vi "VIH HelpGen - Build Progress Info Window.vi"(6 "Mode (run1)":enum16{"start", "stop", "run1", "run2"}(ring)=enum."run1", 7 "Message":string, 8 "error in":errorcluster, 9 "# steps":i32, 10 "step idx":i32=-1, 11 "Cur path":path) -> (0 "error out":errorcluster)   [LabVIEW 2014]
doc: "::: VI Helpeks :::\nCopyright (c) 2000-2026 Konstantin Shifershteyn. All rights reserved."
uses:
  <vilib>/Platform/browser.llb/Open URL in Default Browser (path).vi
panel:
  in  "%OpenHelp":bool caption="Open Built Help"
  in  "%Explore":bool caption="Explore"
  out "errors":string
  in  "%ShowLog":bool caption="Open Build Log"
  out "progress info":string="1 of 1"
  out "Progress bar":i32(slide) scale=0.0..2.0
  out "State":string="Running..."
  out "Current path":string="file path..."
  in  "%Cancel":bool caption="Cancel"
  in  "%DONE":bool caption="Done"
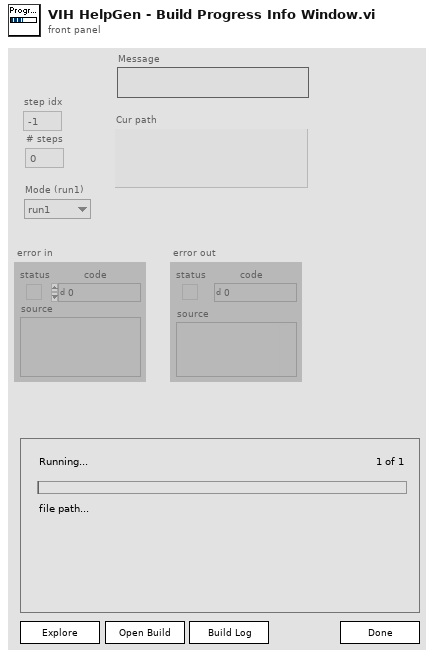
[diagram p1: front panel]
types:
  T1 = cluster{"Common path":path, "HTML File paths":path[], "CHM Path":path}
  T2 = enum8{"Enabled", "Disabled", "Disabled and Grayed Out"}
  T3 = cluster{"Selection Start":i32, "Selection End":i32}
  T4 = cluster{"Show Window":bool, "Show Progress":bool, "Generate HTML":bool, "Generate HHP":bool, "Generate CHM":bool}
  T5 = typedef "eventvkey.ctl" = enum16{"ASCII", "Enter", "Return", "Shift", "Ctrl", "Alt", "Cmd", "Opt", "Caps", "NumLock", "Clear", "Break", "Up", "Down", "Left", "Right", "Insert", "Delete", "Home", "End", "PageUp", "PageDown", "Escape", "Help", "Pause", "ScrollLock", "F1", "F2", "F3", "F4", "F5", "F6", "F7", "F8", "F9", "F10", "F11", "F12", "F13", "F14", "F15", "F16", "F17", "F18", "F19", "F20", "F21", "F22", "F23", "F24", "Play", "VolumeUp", "VolumeDown", "Mute", "Two Byte Char"}
  T6 = cluster{"Shift":bool, "Ctrl":bool, "Alt":bool, "Cmd":bool, "Opt":bool}
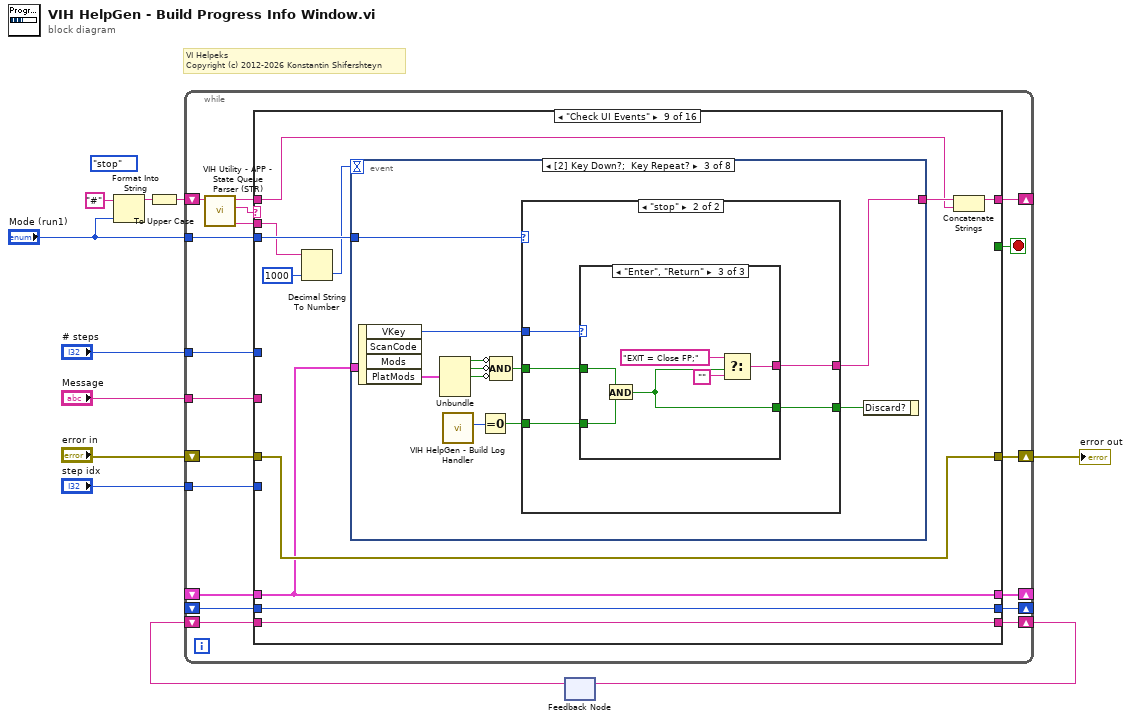
[diagram p0: block diagram]
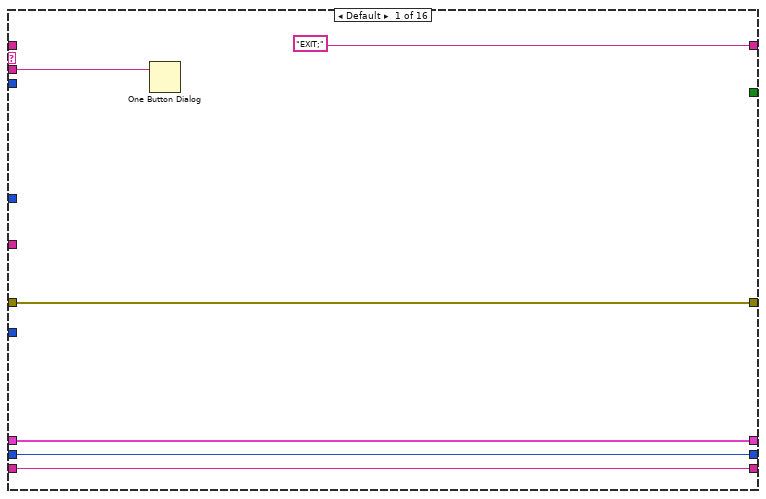
[diagram p2: hidden frame]
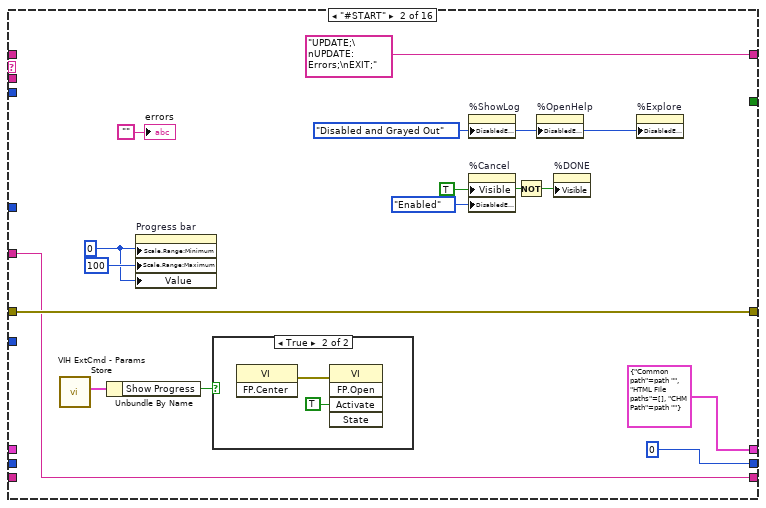
[diagram p3: hidden frame]
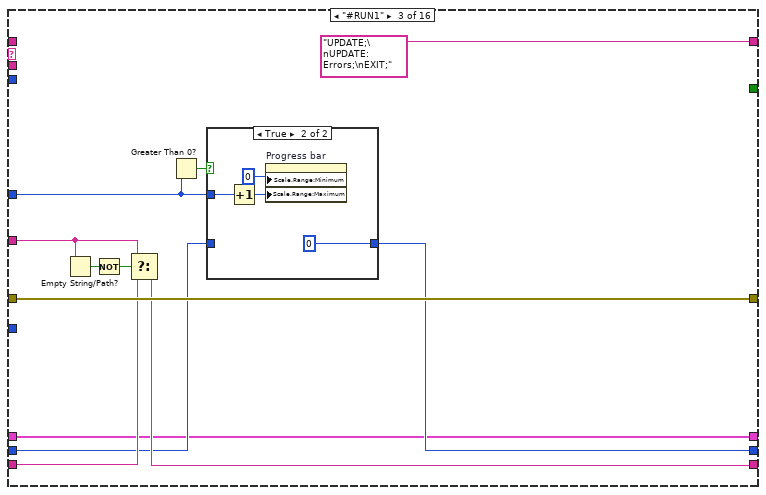
[diagram p5: hidden frame]
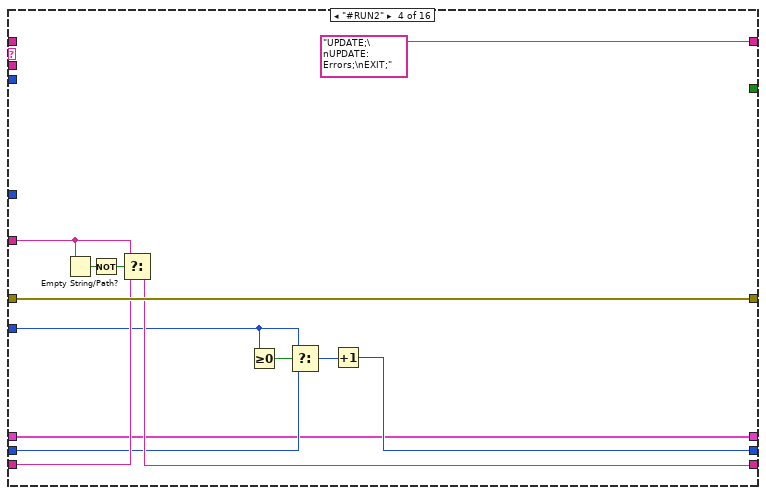
[diagram p7: hidden frame]
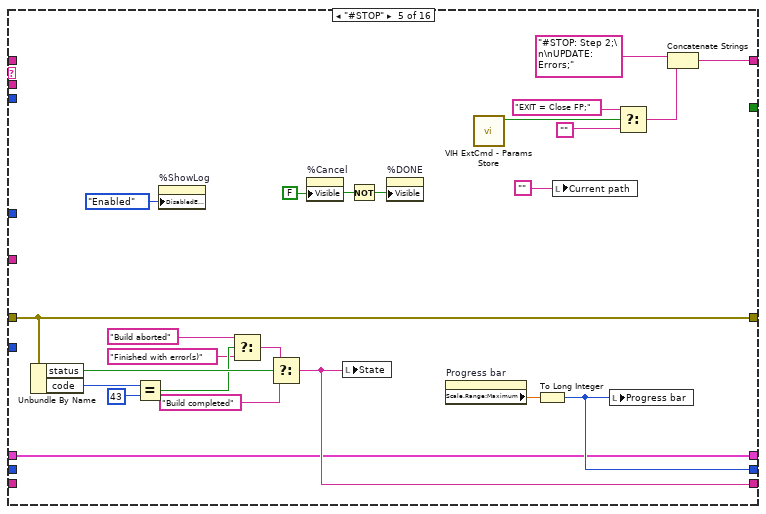
[diagram p8: hidden frame]
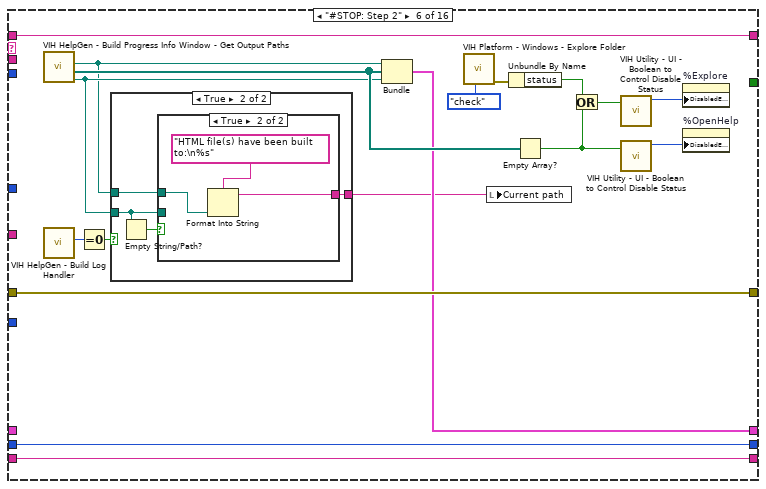
[diagram p9: hidden frame]
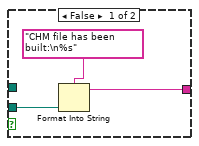
[diagram p11: hidden frame]
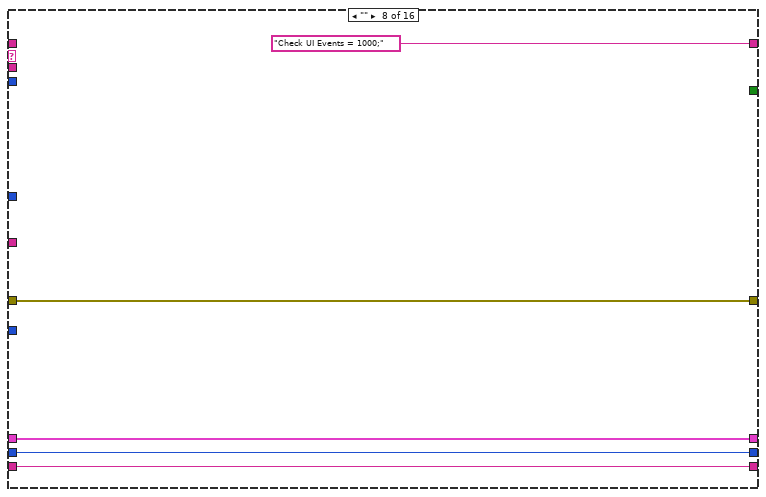
[diagram p13: hidden frame]
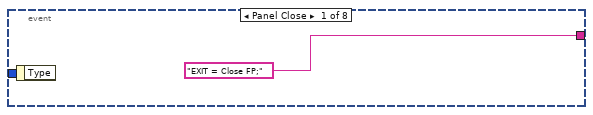
[diagram p14: hidden frame]
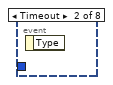
[diagram p15: hidden frame]
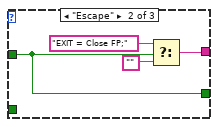
[diagram p18: hidden frame]
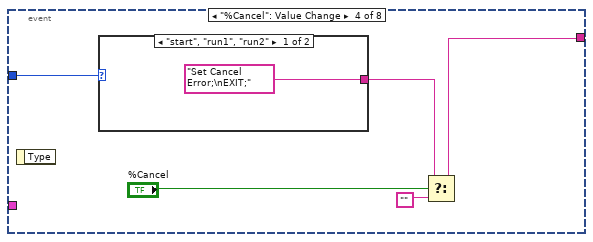
[diagram p19: hidden frame]
diagram:
  (unwired) enum16{"start", "stop", "run1", "run2"}."stop" ("Mode (run1)")
  # "VI Helpeks\nCopyright (c) 2012-2026 Konstantin Shifershteyn"
  n1 = Format Into String(initial string="#", "Mode (run1)") -> (resulting string=w11:string)  [unwired: 2 in, 1 out]
  n2 = To Upper Case(1:w11) -> (0:w7:string)
  n3 = feedback #1() -> (w4:string)  [unwired: 1 in]
  n4 = while {
    shift-right: [w26] -> _
    shift-left: w7 -> [w29]
    shift-right: [w23] -> w9
    shift-left: "error in" -> [w22]
    shift-right: [w20] -> w5
    shift-left: w4 -> [w19]
    tunnel: "Message" -> [w21]
    tunnel: "# steps" -> [w18]
    shift-right: [w17] -> _
    shift-left: _ -> [w16]
    tunnel: "step idx" -> [w15]
    shift-right: [w14] -> _
    shift-left: _ -> [w13]
    tunnel: "Mode (run1)" -> [w12]
    stop <- w25 stop-if-true
    n5 = call "VIH Utility - APP - State Queue Parser (STR).vi"("input queue"=w29) -> ("state parameters"=w27:string, "state"=w28:string, "remained queue"=w24:string)  [unwired: 5 in, 1 out]
    n6 = case shown="\"Check UI Events\"" w28 {
      tunnel: w27 -> [w35 _ _ _ _ _ _ _ w147 _ _ _ _ _ w272 _]
      tunnel: ["EXIT;" "UPDATE;\nUPDATE: Errors;\nEXIT;" "UPDATE;\nUPDATE: Errors;\nEXIT;" "UPDATE;\nUPDATE: Errors;\nEXIT;" w84 w120 w135 "Check UI Events = 1000;" w144 w210 w220 w234 w250 w258 w269 w286] -> w26
      tunnel: [_ _ _ _ _ _ _ _ _ _ _ _ _ _ _ TRUE] -> w25
      tunnel: w24 -> [_ _ _ _ _ w120 w135 _ w143 w210 w220 w234 w250 w258 w275 w286]
      tunnel: [w34 w47 w62 w80 w99 w119 w136 w141 w150 w211 w219 w235 w251 w257 w270 w282] -> w23
      tunnel: w22 -> [w34 w47 w62 w80 w99 w119 w136 w141 w150 w211 w219 w235 w251 w253 w270 w282]
      tunnel: w21 -> [_ w46 w60 w78 _ _ _ _ _ _ _ _ _ _ _ _]
      tunnel: [w32 w46 w57 w75 w95 w122 w137 w142 w153 w212 w216 w237 w252 w256 w274 w285] -> w20
      tunnel: w19 -> [w32 _ w58 w76 _ w122 w137 w142 w153 w212 w216 w237 w252 w256 w274 w285]
      tunnel: w18 -> [_ _ w56 _ _ _ _ _ _ _ _ _ _ _ _ _]
      tunnel: [w31 0 w54 w74 w101 w121 w134 w140 w152 w209 w215 w236 w249 w255 w273 w284] -> w17
      tunnel: w16 -> [w31 _ w53 w73 _ w121 w134 w140 w152 w209 w215 w236 w249 w255 w273 w284]
      tunnel: w15 -> [_ _ _ w71 _ _ _ _ _ _ _ _ _ _ _ _]
      tunnel: [w30 T1 {"Common path"=path "", "HTML File paths"=[], "CHM Path"=path ""} w52 w69 w89 w116 w133 w139 w149 w208 w213 w231 w248 w254 w271 w283] -> w14
      tunnel: w13 -> [w30 _ w52 w69 w89 _ w133 w139 w149 w208 w213 w231 w248 w254 w271 w283]
      tunnel: w12 -> [_ _ _ _ _ _ _ _ w148 _ _ _ _ _ _ _]
      frame Default {
        n7 = One Button Dialog(message=w35) -> ()  [unwired: 1 in, 1 out]
      }
      frame "#START" {
        w43 = TRUE ("Visible")
        w44 = T2."Disabled and Grayed Out" ("Disabled")
        w37 = 0 ("Scale.Range:Minimum")
        n8 = call "VIH ExtCmd - Params Store.vi"() -> ("Params"=w40:T4)  [unwired: 10 in, 1 out]
        n9 = Unbundle By Name(w40) -> ("Show Progress"=w39:bool)
        n10 = property on="Progress bar" class="Slide (strict)"("Scale.Range:Minimum"=w37, "Scale.Range:Maximum"=100, "Value"=w37) -> ()  [unwired: 2 in, 2 out]
        n11 = case shown="True" w39 {
          frame False {
          }
          frame True {
            n12 = invoke class="VI" method="FP.Center"() -> (error out=w51:errorcluster)  [unwired: 3 in, 2 out]
            n13 = invoke class="VI" method="FP.Open"(error in=w51, "Activate"=TRUE ("Activate?")) -> ()  [unwired: 3 in, 5 out]
          }
        }
        n14 = property on="%ShowLog" class="Bool"("DisabledEnum"=w44) -> ()  [unwired: 2 in, 2 out]
        n15 = property on="%Cancel" class="Bool"("Visible"=w43, "DisabledEnum"=T2."Enabled" ("Disabled")) -> ()  [unwired: 2 in, 2 out]
        n16 = Not(x=w43) -> (.not. x?=w42:bool)
        n17 = property on="%OpenHelp" class="Bool"("DisabledEnum"=w44) -> ()  [unwired: 2 in, 2 out]
        n18 = property on="%DONE" class="Bool"("Visible"=w42) -> ()  [unwired: 2 in, 2 out]
        n19 = property on="%Explore" class="Bool"("DisabledEnum"=w44) -> ()  [unwired: 2 in, 2 out]
        "errors" <- ""
      }
      frame "#RUN1" {
        n20 = Empty String/Path?(string/path=w60) -> (empty?=w61:bool)
        n21 = Not(x=w61) -> (.not. x?=w59:bool)
        n22 = Select(t=w60, s=w59, f=w58) -> (s? t:f=w57:string)
        n23 = Greater Than 0?(x=w56) -> (x > 0?=w55:bool)
        n24 = case shown="True" w55 {
          tunnel: w56 -> [_ w67]
          tunnel: [w64 0] -> w54
          tunnel: w53 -> [w64 _]
          frame False {
          }
          frame True {
            n25 = Increment(x=w67) -> (x+1=w65:i32)
            n26 = property on="Progress bar" class="Slide (strict)"("Scale.Range:Minimum"=0, "Scale.Range:Maximum"=w65) -> ()  [unwired: 2 in, 2 out]
          }
        }
      }
      frame "#RUN2" {
        n27 = Empty String/Path?(string/path=w78) -> (empty?=w79:bool)
        n28 = Not(x=w79) -> (.not. x?=w77:bool)
        n29 = Select(t=w78, s=w77, f=w76) -> (s? t:f=w75:string)
        n30 = Greater Or Equal To 0?(x=w71) -> (x >= 0?=w70:bool)
        n31 = Select(t=w71, s=w70, f=w73) -> (s? t:f=w72:i32)
        n32 = Increment(x=w72) -> (x+1=w74:i32)
      }
      frame "#STOP" {
        w88 = FALSE ("Visible")
        n33 = Unbundle By Name(w99) -> ("status"=w94:bool, "code"=w97:i32)
        n34 = Equal?(x=w97, y=43 ("x")) -> (x = y?=w93:bool)
        n35 = property on="%ShowLog" class="Bool"("DisabledEnum"=T2."Enabled" ("Disabled")) -> ()  [unwired: 2 in, 2 out]
        n36 = Select(t="Build aborted", s=w93, f="Finished with error(s)") -> (s? t:f=w92:string)
        n37 = Select(t=w92, s=w94, f="Build completed") -> (s? t:f=w95:string)
        n38 = property on="%Cancel" class="Bool"("Visible"=w88) -> ()  [unwired: 2 in, 2 out]
        n39 = local write "State"(w95) -> ()
        n40 = Not(x=w88) -> (.not. x?=w87:bool)
        n41 = property on="%DONE" class="Bool"("Visible"=w87) -> ()  [unwired: 2 in, 2 out]
        n42 = property on="Progress bar" class="Slide (strict)"() -> ("Scale.Range:Maximum"=w104:dbl)  [unwired: 2 in, 2 out]
        n43 = call "VIH ExtCmd - Params Store.vi"() -> ("Ext Command"=w86:bool)  [unwired: 10 in, 1 out]
        n44 = To Long Integer(number=w104) -> (32bit integer=w101:i32)
        n45 = local write "Current path"("") -> ()
        n46 = local write "Progress bar"(w101) -> ()
        n47 = Select(t="EXIT = Close FP;", s=w86, f="") -> (s? t:f=w83:string)
        n48 = Concatenate Strings("#STOP: Step 2;\n\nUPDATE: Errors;", w83) -> (w84:string)
      }
      frame "#STOP: Step 2" {
        n49 = call "VIH HelpGen - Build Progress Info Window - Get Output Paths.vi"() -> ("CHM Path"=w107:path, "HTML File paths"=w117:path[], "Common path"=w105:path)  [unwired: 9 in]
        n50 = call "VIH HelpGen - Build Log Handler.vi"() -> ("errors"=w109:i32)  [unwired: 7 in, 4 out]
        n51 = Equal To 0?(x=w109) -> (x = 0?=w108:bool)
        n52 = case shown="True" w108 {
          tunnel: w107 -> [_ w125]
          tunnel: [_ w124] -> w106
          tunnel: w105 -> [_ w123]
          frame False {
          }
          frame True {
            n53 = Empty String/Path?(string/path=w125) -> (empty?=w126:bool)
            n54 = case shown="True" w126 {
              tunnel: w125 -> [w129 _]
              tunnel: [w127 w131] -> w124
              tunnel: w123 -> [_ w130]
              frame False {
                n55 = Format Into String(format string="CHM file has been built:\n%s", w129) -> (resulting string=w127:string)  [unwired: 2 in, 1 out]
              }
              frame True {
                n56 = Format Into String(format string="HTML file(s) have been built to:\n%s", w130) -> (resulting string=w131:string)  [unwired: 2 in, 1 out]
              }
            }
          }
        }
        n57 = Bundle("Common path"=w105, "HTML File paths"=w117, "CHM Path"=w107) -> (w116:T1)  [unwired: 1 in]
        n58 = call "VIH Platform - Windows - Explore Folder.vi"("cmd (run)"=enum16{"run", "check"}."check") -> ("error out"=w114:errorcluster)  [unwired: 10 in]
        n59 = local write "Current path"(w106) -> ()
        n60 = Unbundle By Name(w114) -> ("status"=w113:bool)
        n61 = Empty Array?(array=w117) -> (empty?=w112:bool)
        n62 = Or(x=w113, y=w112) -> (x .or. y?=w111:bool)
        n63 = call "VIH Utility - UI - Boolean to Control Disable Status.vi"("Status in"=w111) -> ("Control Disable if True"=w110:u8)  [unwired: 3 in, 1 out]
        n64 = call "VIH Utility - UI - Boolean to Control Disable Status.vi"("Status in"=w112) -> ("Control Disable if True"=w118:u8)  [unwired: 3 in, 1 out]
        n65 = property on="%Explore" class="Bool"("DisabledEnum"=w110) -> ()  [unwired: 2 in, 2 out]
        n66 = property on="%OpenHelp" class="Bool"("DisabledEnum"=w118) -> ()  [unwired: 2 in, 2 out]
      }
      frame "--------------------------- 1" {
      }
      frame "" {
      }
      frame "Check UI Events" {
        n67 = Decimal String To Number(string=w147, default (0L)=1000 ("default (0 I32)")) -> (number=w146:i32)  [unwired: 1 in, 1 out]
        n68 = event shown="[2] Key Down?;  Key Repeat?" {
          selector: _ -> [_ _ _ _ _ _ _ _]
          dyn-events: _ -> [_ _ _ _ _ _ _ _]
          timeout: w146 -> [_ _ _ _ _ _ _ _]
          tunnel: ["EXIT = Close FP;" _ w165 w181 "EXIT = Close FP;" _ _ _] -> w151
          tunnel: w149 -> [_ _ _ _ _ _ w195 w207]
          tunnel: w148 -> [_ _ w157 w185 _ _ _ _]
          event Panel Close {
            n69 = event-data() -> ()  [unwired: 1 in, 1 out]
          }
          event Timeout {
            n70 = event-data() -> ()  [unwired: 1 in, 1 out]
          }
          event Key Down?; event type 5.0.x8000000b {
            n71 = event-data() -> ("VKey"=w164:T5, "PlatMods"=w163:T6)  [unwired: 1 in, 2 out]
            n72 = Unbundle(w163) -> ("Shift"=w162:bool, "Ctrl"=w161:bool, "Alt"=w160:bool)  [unwired: 2 out]
            n73 = call "VIH HelpGen - Build Log Handler.vi"() -> ("errors"=w156:i32)  [unwired: 7 in, 4 out]
            n74 = Equal To 0?(x=w156) -> (x = 0?=w155:bool)
            n75 = Compound Arithmetic op=AND(invert w162, invert w161, invert w160) -> (w159:bool)
            n76 = case shown="\"stop\"" w157 {
              tunnel: [_ w170] -> w165
              tunnel: w164 -> [_ w169]
              tunnel: w159 -> [_ w168]
              tunnel: [_ w167] -> w158
              tunnel: w155 -> [_ w166]
              frame Default {
              }
              frame "stop" {
                n77 = case shown="\"Enter\", \"Return\"" w169 {
                  tunnel: [_ w172 w178] -> w170
                  tunnel: w168 -> [_ w171 w177]
                  tunnel: [_ w171 w175] -> w167
                  tunnel: w166 -> [_ _ w176]
                  frame Default {
                  }
                  frame "Escape" {
                    n78 = Select(t="EXIT = Close FP;", s=w171, f="") -> (s? t:f=w172:string)
                  }
                  frame "Enter", "Return" {
                    n79 = And(x=w177, y=w176) -> (x .and. y?=w175:bool)
                    n80 = Select(t="EXIT = Close FP;", s=w175, f="") -> (s? t:f=w178:string)
                  }
                }
              }
            }
            n81 = event-data("Discard?"=w158) -> ()  [unwired: 1 in, 1 out]
          }
          event "%Cancel": Value Change {
            n82 = event-data() -> ()  [unwired: 1 in, 1 out]
            n83 = case shown="\"start\", \"run1\", \"run2\"" w185 {
              tunnel: ["Set Cancel Error;\nEXIT;" _] -> w183
              frame "start", "run1", "run2" {
              }
              frame "stop" {
              }
            }
            n84 = Select(t=w183, s="%Cancel", f="") -> (s? t:f=w181:string)
          }
          event "%DONE": Value Change {
            n85 = event-data() -> ()  [unwired: 1 in, 1 out]
          }
          event "%ShowLog": Value Change {
            n86 = event-data() -> ()  [unwired: 1 in, 1 out]
            n87 = call "VIH HelpGen - Build Log Handler.vi"() -> ("log file path"=w189:path)  [unwired: 7 in, 4 out]
            n88 = call-poly <vilib>:"Open URL in Default Browser.vi"("path"=w189) -> ("error out"=w188:errorcluster)  [unwired: 5 in, 1 out]
            n89 = call <vilib>:"Simple Error Handler.vi"("error in (no error)"=w188) -> ()  [unwired: 4 in, 5 out]
          }
          event "%OpenHelp": Value Change {
            n90 = event-data() -> ()  [unwired: 1 in, 1 out]
            n91 = Unbundle(w195) -> ("HTML File paths"=w194:path[], "CHM Path"=w190:path)  [unwired: 1 out]
            n92 = Index Array(array=w194) -> (element=w192:path)  [unwired: 1 in]
            n93 = Empty String/Path?(string/path=w190) -> (empty?=w191:bool)
            n94 = case shown="True" w191 {
              tunnel: [w196 w199] -> w193
              tunnel: w192 -> [_ w198]
              tunnel: w190 -> [w197 _]
              frame False {
                n95 = call "VIH Utility - HELP - Open Help File.vi"("Help Path"=w197) -> ("error out"=w196:errorcluster)  [unwired: 9 in, 1 out]
              }
              frame True {
                n96 = call-poly <vilib>:"Open URL in Default Browser.vi"("path"=w198) -> ("error out"=w199:errorcluster)  [unwired: 5 in, 1 out]
              }
            }
            n97 = call <vilib>:"Simple Error Handler.vi"("error in (no error)"=w193) -> ()  [unwired: 4 in, 5 out]
          }
          event "%Explore": Value Change {
            n98 = event-data() -> ()  [unwired: 1 in, 1 out]
            n99 = Unbundle(w207) -> ("Common path"=w201:path, "CHM Path"=w202:path)  [unwired: 1 out]
            n100 = Empty String/Path?(string/path=w202) -> (empty?=w204:bool)
            n101 = Strip Path(path=w202) -> (stripped path=w203:path)  [unwired: 1 out]
            n102 = Select(t=w201, s=w204, f=w203) -> (s? t:f=w200:path)
            n103 = call "VIH Platform - Windows - Explore Folder.vi"("cmd (run)"=enum16{"run", "check"}."run", "exe/doc/dir path"=w200) -> ("error out"=w205:errorcluster)  [unwired: 9 in]
            n104 = call <vilib>:"Simple Error Handler.vi"("error in (no error)"=w205) -> ()  [unwired: 4 in, 5 out]
          }
        }
        n105 = Concatenate Strings(w151, w143) -> (w144:string)
      }
      frame "--------------------------- 2" {
      }
      frame "UPDATE" {
        n106 = case shown="1.." w215 {
          selector: w215 -> [_ w223]
          tunnel: [_ w222] -> w214
          frame ..0 {
          }
          frame 1.. {
            n107 = property on="Progress bar" class="Slide (strict)"() -> ("Scale.Range:Maximum"=w225:dbl)  [unwired: 2 in, 2 out]
            n108 = Decrement(x=w225) -> (x-1=w221:dbl)
            n109 = Format Into String(format string="%d of %d", w223, w221) -> (resulting string=w222:string)  [unwired: 2 in, 1 out]
          }
        }
        "progress info" <- w214
        n110 = Path To String(path="Cur path") -> (string=→"Current path":string)
        "State" <- w216
        "Progress bar" <- w215
      }
      frame "UPDATE: Errors" {
        n111 = property on="errors" class="Str"("Value"="", "Text.Selection"=T3 {"Selection Start"=0, "Selection End"=-1}, "Text.FontBold"=TRUE ("Text.Font:Bold"), "Text.FontColor"=u32 16711680) -> (error out=w226:errorcluster)  [unwired: 2 in, 1 out]
        n112 = call "VIH HelpGen - Build Log Handler.vi"() -> ("errors"=w232:i32)  [unwired: 7 in, 4 out]
        n113 = Greater Than 0?(x=w232) -> (x > 0?=w233:bool)
        n114 = case shown="True" w233 {
          tunnel: w232 -> [_ w247]
          tunnel: w226 -> [_ _]
          frame False {
          }
          frame True {
            n115 = Format Into String(format string="Errors:  %d", w247) -> (resulting string=w244:string)  [unwired: 2 in, 1 out]
            n116 = Concatenate Strings(w244, "  [view the Build Log for details]" ("format string")) -> (w239:string)
            n117 = String Length(string=w244) -> (length=w238:i32)
            n118 = Bundle(w238, -1) -> (w241:cluster{i32, i32})  [unwired: 1 in]
            n119 = property on="errors" class="Str"("Value"=w239, "Text.Selection"=w241, "Text.FontBold"=FALSE, "Text.FontColor"=u32 0) -> ()  [unwired: 2 in, 2 out]
          }
        }
      }
      frame "--------------------------- 3" {
      }
      frame "Set Cancel Error" {
        n120 = case shown="No Error" w253 {
          selector: w253 -> [w259 w266]
          tunnel: [w263 w266] -> w257
          frame No Error {
            n121 = disable-structure shown="Enabled" {
              disable-tunnel: [w264 "Build help files"] -> w260
              frame Disabled {
                n122 = property class="VI"() -> ("Name"=w264:string)  [unwired: 2 in, 2 out]
              }
              frame Enabled {
              }
            }
            n123 = Bundle By Name(cluster=w259, "status"=TRUE, "code"=43, "source"=w260) -> (w263:errorcluster)
          }
          frame Error {
          }
        }
      }
      frame "EXIT" {
        n124 = case shown="\"Close FP\"" w272 {
          tunnel: ["Check UI Events = 5;" _] -> w267
          frame Default {
          }
          frame "Close FP" {
            n125 = property on="errors" class="Str"("Value"="", "Text.Selection"=T3 {"Selection Start"=0, "Selection End"=-1}, "Text.FontBold"=TRUE ("Text.Font:Bold"), "Text.FontColor"=u32 16711680) -> ()  [unwired: 2 in, 2 out]
            n126 = invoke class="VI" method="FP.Close"() -> ()  [unwired: 3 in, 3 out]
            n127 = property on="Progress bar" class="Slide (strict)"("Value"=0 ("Progress bar")) -> ()  [unwired: 2 in, 2 out]
          }
        }
        n128 = Concatenate Strings(w267, "HALT;", w275) -> (w269:string)
      }
      frame "HALT" {
      }
    }
  }
  "error out" <- w9
  n129 = feedback-in #1(w5) -> ()
